vi "Get Command Bits.vi"(8 "error in (no error)":errorcluster, 11 "RFFE Command in":refnum<class "RFFE Command.lvclass">) -> (0 "error out":errorcluster, 2 "Command Bits":u8[](array[numeric]) format="%02x", 3 "RFFE Command out":refnum<class "RFFE Command.lvclass">)   [LabVIEW 2018, in "MIPI RFFE API.lvlib" / "RFFE Command.lvclass"]
uses:
  RFFE Command.lvclass
  MIPI RFFE API.lvlib
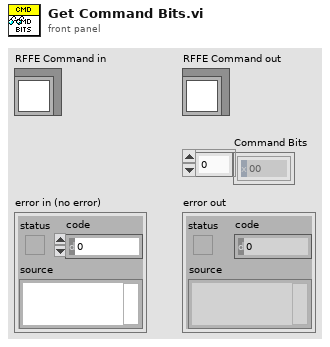
[diagram p1: front panel]
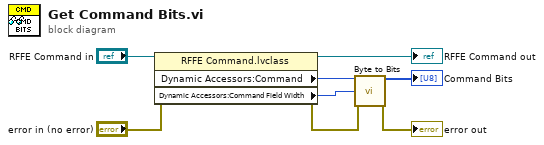
[diagram p0: block diagram]
diagram:
  n1 = property class="RFFE Command.lvclass"(reference="RFFE Command in", error in="error in (no error)") -> (reference out=→"RFFE Command out":refnum<class "RFFE Command.lvclass">, error out=w4:errorcluster, "Dynamic Accessors:Command"=w7:u8, "Dynamic Accessors:Command Field Width"=w6:i32)
  n2 = call "Byte to Bits.vi"("Byte"=w7, "Bit Width"=w6, "error in (no error)"=w4) -> ("Bits"=→"Command Bits":u8[], "error out"=→"error out":errorcluster)  [unwired: 11 in]
